vi "UI Subpanel.vi"() -> ()   [LabVIEW 2021, in "CIF CAN_Reader_CANsub UI.lvlib"]
uses:
  CIF CAN_Reader_CANsub UI.lvlib
  Common/Typedef/Configuration.ctl
  <vilib>/CIF Foundation/CIF Core/CIFCore/Common/Typedef/Common Plugin Configuration.ctl
  <vilib>/CIF Foundation/CIF Core/CIFCore/Common/Typedef/External Clock Config.ctl
  <vilib>/CIF Foundation/CIF CAN RW Core/typedef/CAN Port Configuration.ctl
  <vilib>/CIF Foundation/CIF CAN RW Core/typedef/CAN Mode.ctl
  <vilib>/CIF Foundation/CIF CAN RW Core/typedef/FD Config.ctl
  <vilib>/CIF Foundation/CIF CAN RW Core/typedef/CAN Filter.ctl
  <vilib>/CIF Foundation/CIF Core/CIFUI/Typedef/Class Data for SubPanel.ctl
  <vilib>/CIF Foundation/CIF Core/CIFUI/Typedef/Core UI References.ctl
  <vilib>/CIF Foundation/CIF Core/CIFUI/Typedef/Run Listen Button.ctl
  <vilib>/CIF Foundation/CIF Core/CIFUI/Typedef/SubPanel Events.ctl
  <vilib>/CIF Foundation/CIF Core/CIFUI/Typedef/New Connection Plugin Event Data.ctl
  Grpc/CanReaderCansub_client/RPC Messages/cif_can_reader_cansub_Statistics.ctl
  <vilib>/CIF Foundation/CIF CAN RW Core/typedef/CAN Status.ctl
  <vilib>/CIF Foundation/CIF CAN RW Core/typedef/Communication State.ctl
  <vilib>/CIF Foundation/CIF CAN RW Core/typedef/Last Error.ctl
  <vilib>/CIF Foundation/CIF Core/CIFUI/CIF_UI.lvclass
  <vilib>/CIF Foundation/CIF Core/CIFUI/CIF_UI.lvclass/CIF_UI.ctl
  <vilib>/CIF Foundation/CIF U8 Array Monitor gRPC/U8_Array_Monitor_gRPC/CIFU8ArrayMonitor_client/RPC Messages/cif_u8arraymonitor_SetEnableU8ArrayRequest.ctl
  <vilib>/CIF Foundation/CIF Core/CIFUI/Utilities/Get Human Readable Error.vi
  <vilib>/CIF Foundation/CIF Utilities/Errors/Append Error Location.vi
  <vilib>/CIF Foundation/CIF Utilities/Errors/Human Readable Error Message.vi
  Grpc/CAN_Reader_CANsub_wrapper/CAN_Reader_CANsub_Wrapper.lvlib
  <vilib>/addons/_JKI.lib/Serialization/JSON/JKI JSON Serialization.lvlib
  <vilib>/CIF Foundation/CIF Core/CIFCore/Grpc/CIFCoreWrapper/CIFCoreWrapper.lvlib
  <vilib>/CIF Foundation/CIF U8 Array Monitor gRPC/U8_Array_Monitor_gRPC/CIFU8ArrayMonitorWrapper/CIFU8ArrayMonitorWrapper.lvlib
  <vilib>/CIF Foundation/CIF U8 Array Monitor gRPC/U8_Array_Monitor_gRPC/CIFU8ArrayMonitor_client/CIFU8ArrayMonitor_client.lvlib
  <vilib>/CIF Foundation/CIF Core/CIFCore/Common/CIFCoreCommon.lvlib
  Common/CAN_Reader_CANsub_Common.lvlib
  <vilib>/CIF Foundation/CIF CAN RW Core/CAN_RW_CORE.lvclass
  Grpc/CanReaderCansub_client/CanReaderCansub_client.lvlib
panel:
  in  "Blink":bool
  in  "Refresh Device List":bool
  in  "Get CAN Data":bool
  in  "History":u32=10
  in  "Enable CAN Monitor":bool
  in  "Update Config":bool
  out "CAN Status":T1
  out "Devices":string[](array[string])
  out "Statistics":T4
  in  "Class Data for SubPanel":T5
  in  "Configuration":T8={"Common"={"Period (s)"=0.001, "Offset (us)"=0, "Priority"=100, "Processor"=-2, "External Clock"={"ClockID"=0, "Clock Name"="", "Publish Clock"=FALSE, "Convert Data Timestamps"=FALSE, "Plugin Timing Source"=FALSE}}, "RX Interface"="CAN2", "Port Configuration"={"Mode"=enum."CAN FD", "Baud Rate"=500000, "Temination On"=TRUE, "Subordinate"=FALSE, "Echo TX"=FALSE, "FD Config"={"FD Baud Rate"=2000000, "ISO Mode"=TRUE, "BRS Enabled"=TRUE}}, "Timeout (ms)"=100, "Frames to read"=100, "Filter"={"Allow List (ID)"=[], "Deny List (ID)"=[]}} {"Filter"."Deny List (ID)" format="%.0x"; "Filter"."Allow List (ID)" format="%.0x"; "Port Configuration"."FD Config"."FD Baud Rate" format="%.0p"; "Port Configuration"."Baud Rate" format="%.0p"; "Common"."Period (s)" format="%#_13g"}
  out "Plugin Status":string[][](table)
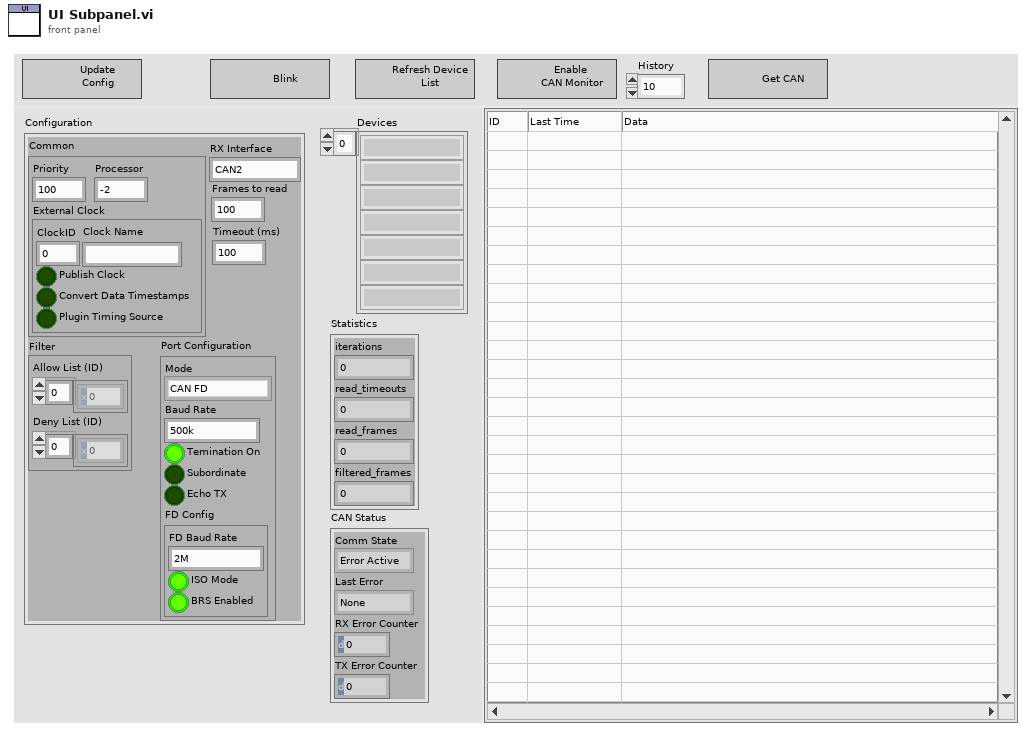
[diagram p1: front panel]
types:
  T1 = typedef "CAN_RW_CORE.lvclass/CAN Status.ctl" = cluster{"Comm State":T2, "Last Error":T3, "RX Error Counter":u8, "TX Error Counter":u8}
  T2 = typedef "CAN_RW_CORE.lvclass/Communication State.ctl" = enum16{"Error Active", "Error Passive", "Bus Off"}
  T3 = typedef "CAN_RW_CORE.lvclass/Last Error.ctl" = enum16{"None", "Stuff", "Form", "Ack", "Bit1", "Bit0", "CRC", "Unknown"}
  T4 = typedef "CanReaderCansub_client.lvlib/cif_can_reader_cansub_Statistics.ctl" = cluster{"iterations":u64, "read_timeouts":u64, "read_frames":u64, "filtered_frames":u64}
  T5 = typedef "CIF_UI.lvclass/Class Data for SubPanel.ctl" = cluster{"IP Address":string, "Server Certificate File (.crt)":path, "Connected":bool, "Core UI References":T6, "Subpanel Events":T7, "Manager gRPC Port":u16}
  T6 = typedef "CIF_UI.lvclass/Core UI References.ctl" = cluster{"Plugin Status":refnum<vi>, "Plugin Status Valid":bool, "Connection":refnum<vi>, "Connection Valid":bool, "Exit":refnum<vi>, "Exit Valid":bool, "Run Listen":refnum<vi>, "Run Listen Valid":bool, "Clear Local Error":refnum<vi>, "Clear Local Error Valid":bool, "Local Error":refnum<vi>, "Local Error Valid":bool}
  T7 = typedef "CIF_UI.lvclass/SubPanel Events.ctl" = cluster{"Clear Local Error":refnum<user-event>, "Shutdown":refnum<user-event>, "Plugin Connection":refnum<user-event>}
  T8 = typedef "CAN_Reader_CANsub_Common.lvlib/Configuration.ctl" = cluster{"Common":T9, "RX Interface":string, "Port Configuration":T11, "Timeout (ms)":i32, "Frames to read":i32, "Filter":T14}
  T9 = typedef "CIFCoreCommon.lvlib/Common Plugin Configuration.ctl" = cluster{"Period (s)":dbl, "Offset (us)":i32, "Priority":i32, "Processor":i32, "External Clock":T10}
  T10 = typedef "CIFCoreCommon.lvlib/External Clock Config.ctl" = cluster{"ClockID":u8, "Clock Name":string, "Publish Clock":bool, "Convert Data Timestamps":bool, "Plugin Timing Source":bool}
  T11 = typedef "CAN_RW_CORE.lvclass/CAN Port Configuration.ctl" = cluster{"Mode":T12, "Baud Rate":u64, "Temination On":bool, "Subordinate":bool, "Echo TX":bool, "FD Config":T13}
  T12 = typedef "CAN_RW_CORE.lvclass/CAN Mode.ctl" = enum16{"CAN 2.0", "CAN FD"}
  T13 = typedef "CAN_RW_CORE.lvclass/FD Config.ctl" = cluster{"FD Baud Rate":u64, "ISO Mode":bool, "BRS Enabled":bool}
  T14 = typedef "CAN_RW_CORE.lvclass/CAN Filter.ctl" = cluster{"Allow List (ID)":u32[], "Deny List (ID)":u32[]}
  T15 = typedef "grpc-lvsupport-release.lvlib/grpcId.ctl" = u64
  T16 = typedef "CIFU8ArrayMonitor_client.lvlib/cif_u8arraymonitor_SetEnableU8ArrayRequest.ctl" = cluster{"enable_u8_array":bool, "history_depth":u32}
  T17 = typedef "CanReaderCansub_client.lvlib/cif_can_reader_cansub_CansubDevice.ctl" = cluster{"interface":string, "slot":u32, "device_id":string}
  T18 = typedef "CAN_Reader_NIXNET_Common.lvlib/Configuration.ctl" = cluster{"Common":T9, "RX Interface":string, "Port Configuration":T11, "Timeout (ms)":i32, "Frames to read":i32, "Filter":T14}
  T19 = typedef "CIFU8ArrayMonitor_client.lvlib/cif_u8arraymonitor_U8Arrays.ctl" = cluster{"u8_array":T20[], "valid":bool}
  T20 = typedef "CIFU8ArrayMonitor_client.lvlib/cif_u8arraymonitor_U8Array.ctl" = cluster{"u8_array":u8[], "timestamp":i64}
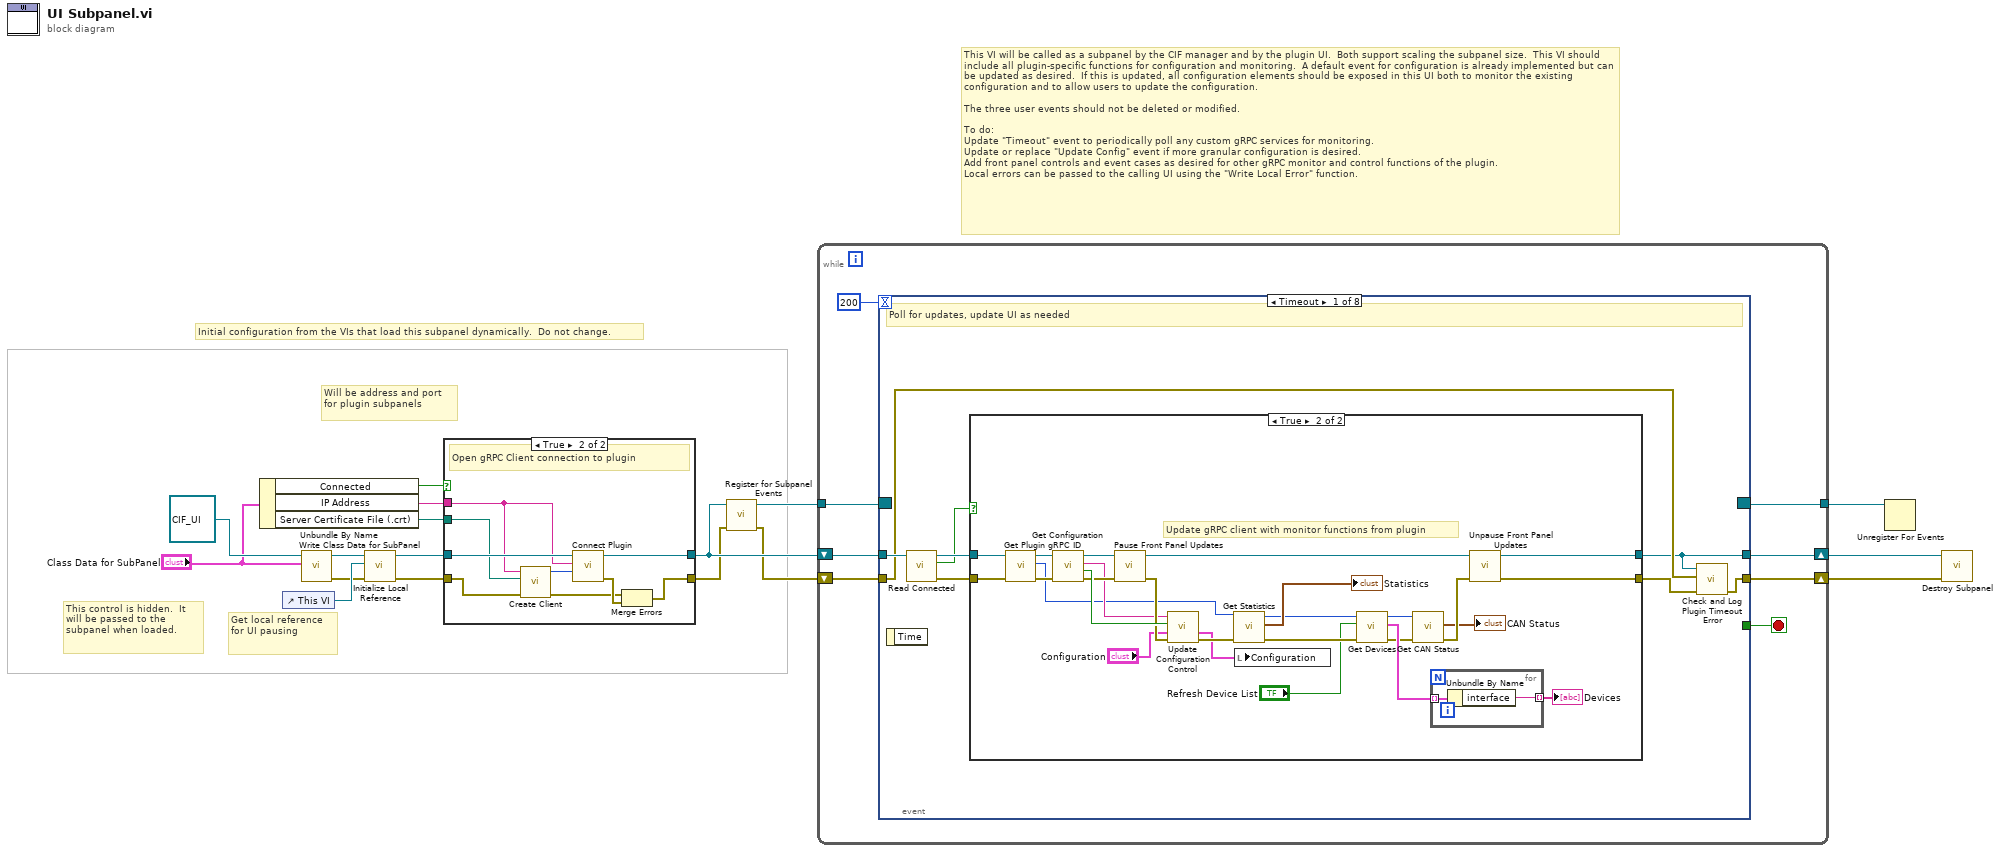
[diagram p0: block diagram]
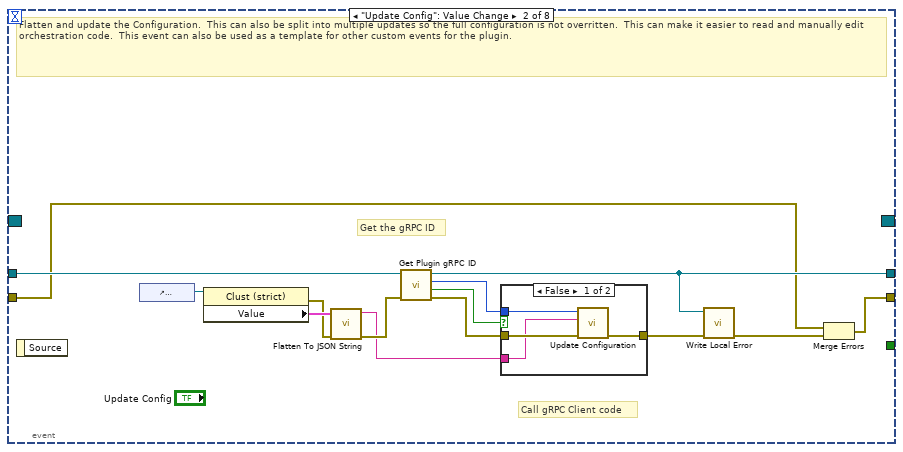
[diagram p4: hidden frame]
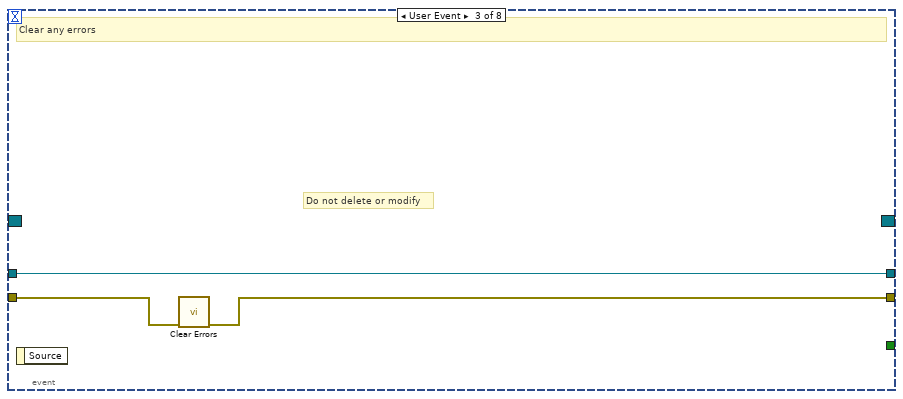
[diagram p6: hidden frame]
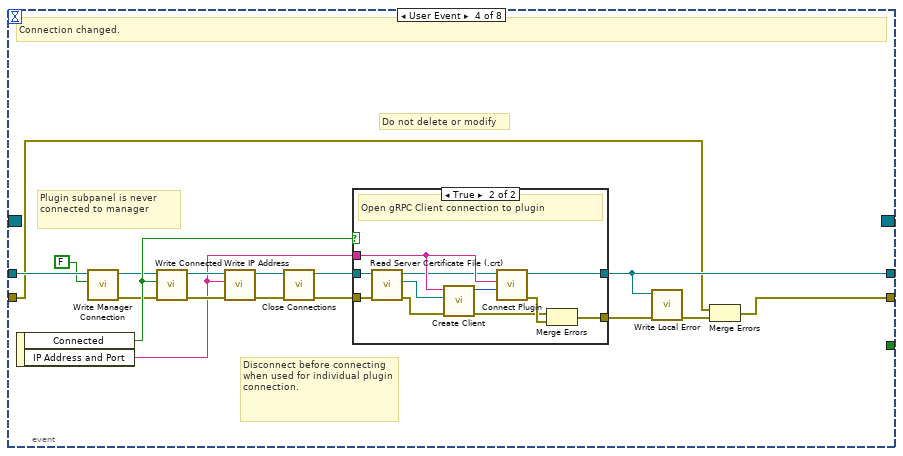
[diagram p7: hidden frame]
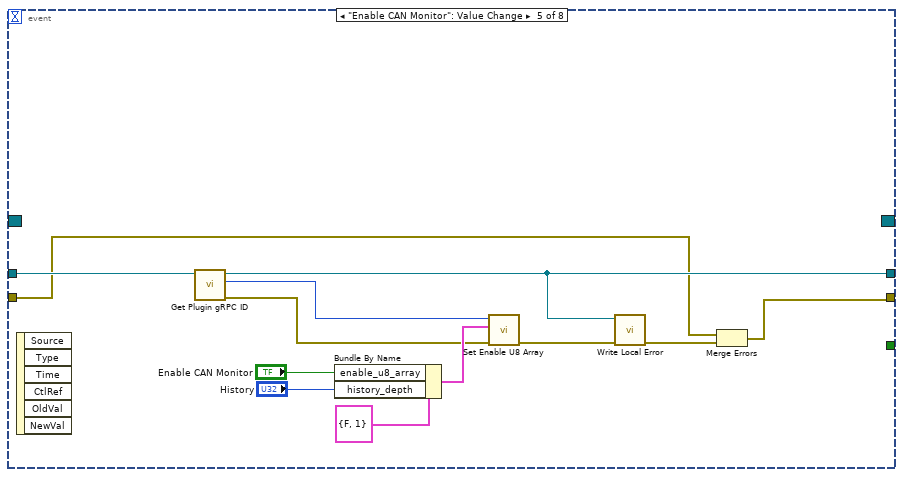
[diagram p9: hidden frame]
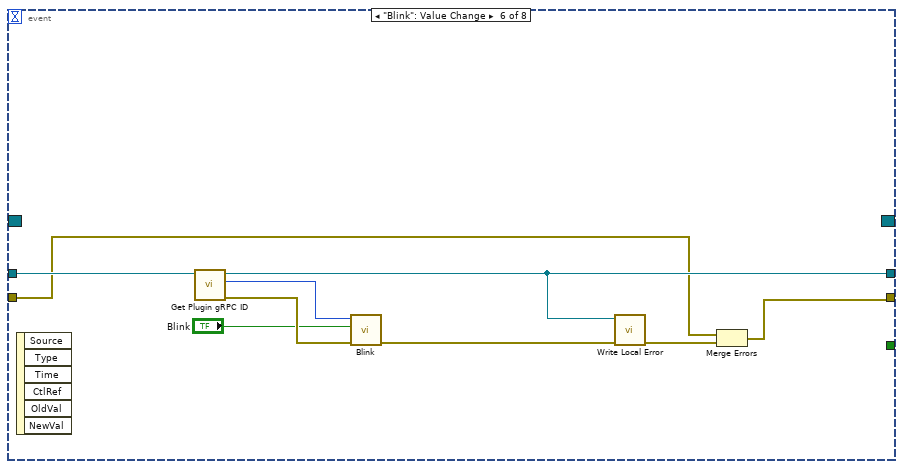
[diagram p10: hidden frame]
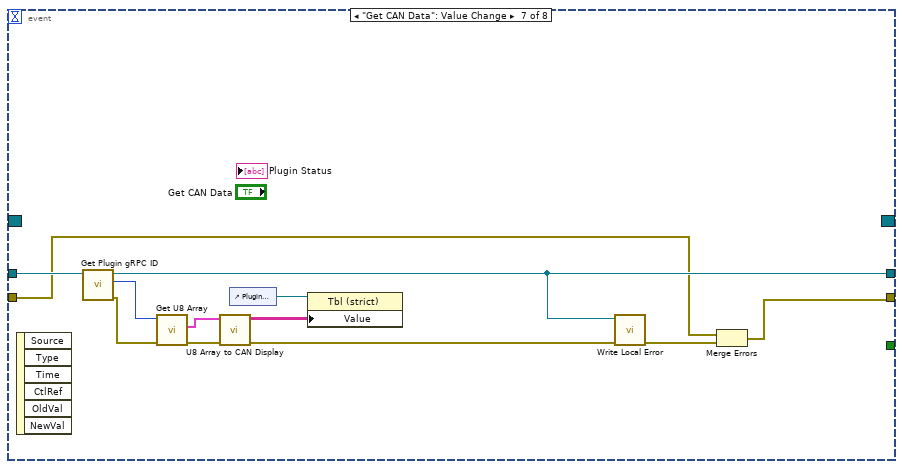
[diagram p11: hidden frame]
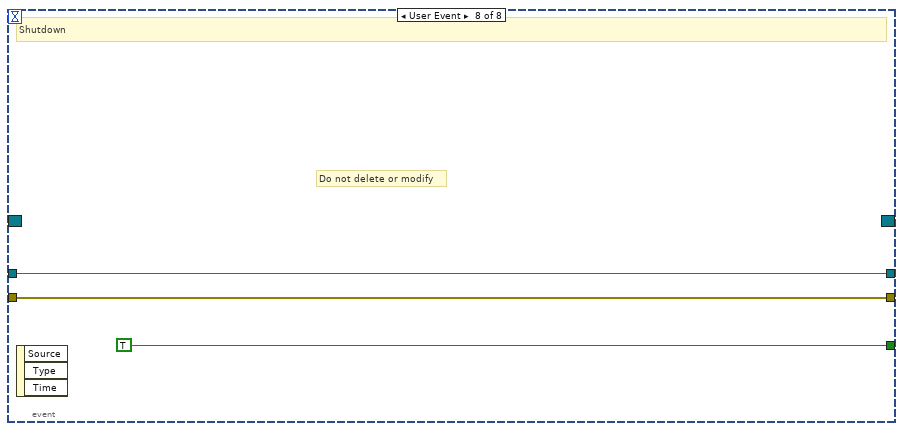
[diagram p12: hidden frame]
diagram:
  # "Initial configuration from the VIs that load this subpanel dynamically.  Do not change."
  # "This control is hidden.  It will be passed to the subpanel when loaded."
  # "This VI will be called as a subpanel by the CIF manager and by the plugin UI.  Both support scaling the subpanel size.  This VI should include all plugin-specific functions for configuration and monitoring.  A default event for configuration is already implemented but can be updated as desired.  If this is updated, all configuration elements should be exposed in this UI both to monitor the existing configuration and to allow users to update the configuration.\n\nThe three user events should not be deleted or modified.\n\nTo do:\nUpdate \"Timeout\" event to periodically poll any custom gRPC services for monitoring.\nUpdate or replace \"Update Config\" event if more granular configuration is desired.\nAdd front panel controls and event cases as desired for other gRPC monitor and control functions of the plugin.\nLocal errors can be passed to the calling UI using the \"Write Local Error\" function."
  # "Will be address and port for plugin subpanels"
  # "Get local reference for UI pausing"
  n1 = Unbundle By Name("Class Data for SubPanel") -> ("Connected"=w8:bool, "IP Address"=w7:string, "Server Certificate File (.crt)"=w6:path)
  n2 = control-ref of="This VI"() -> (w17:refnum<vi>)
  n3 = call <vilib>:"Write Class Data for SubPanel.vi"("Class Data for SubPanel"="Class Data for SubPanel", "CIF_UI in"=refnum<class "CIF_UI.lvclass"> refnum) -> ("error out"=w12:errorcluster, "CIF_UI out"=w14:refnum<class "CIF_UI.lvclass">)  [unwired: 8 in]
  n4 = call <vilib>:"Initialize Local Reference.vi"("error in (no error)"=w12, "This VI"=w17, "CIF_UI in"=w14) -> ("error out"=w10:errorcluster, "CIF_UI out"=w11:refnum<class "CIF_UI.lvclass">)  [unwired: 7 in]
  n5 = case shown="True" w8 {
    tunnel: [w18 w28] -> w4
    tunnel: [w19 w26] -> w5
    tunnel: w11 -> [w19 w25]
    tunnel: w10 -> [w18 w24]
    tunnel: w7 -> [_ w21]
    tunnel: w6 -> [_ w20]
    frame False {
    }
    frame True {
      # "Open gRPC Client connection to plugin"
      n6 = call "Create Client.vi"("error in"=w24, "Server Certificate File (.crt)"=w20, "address"=w21) -> ("error out"=w23:errorcluster, "gRPC ID Out"=w22:T15)  [unwired: 7 in]
      n7 = call <vilib>:"Connect Plugin.vi"("gRPC ID"=w22, "Address"=w21, "CIF_UI in"=w25) -> ("error out"=w27:errorcluster, "CIF_UI out"=w26:refnum<class "CIF_UI.lvclass">)  [unwired: 7 in]
      n8 = Merge Errors(w23, w27) -> (w28:errorcluster)
    }
  }
  n9 = call <vilib>:"Register for Subpanel Events.vi"("error in (no error)"=w4, "CIF_UI in"=w5) -> ("error out"=w2:errorcluster, "Event Registration Refnum"=w3:refnum<event-registration>)  [unwired: 8 in]
  n10 = while {
    tunnel: w3 -> [w35]
    shift-right: [w30] -> w16
    shift-left: w5 -> [w33]
    shift-right: [w31] -> w1
    shift-left: w2 -> [w32]
    tunnel: [w29] -> w15
    stop <- w34 stop-if-true
    n11 = event shown="[0] Timeout" {
      selector: w35 -> [_ _ _ _ _ _ _ _]
      dyn-events: [_ _ _ _ _ _ _ _] -> w29
      timeout: 200 -> [_ _ _ _ _ _ _ _]
      tunnel: [_ _ _ _ _ _ _ TRUE] -> w34
      tunnel: w33 -> [w41 w85 w94 w105 w137 w146 w158 w161]
      tunnel: w32 -> [w38 w79 w96 w98 w135 w144 w156 w160]
      tunnel: [w39 w78 w95 w97 w134 w143 w155 w160] -> w31
      tunnel: [w37 w81 w94 w99 w136 w145 w157 w161] -> w30
      event Timeout {
        # "Poll for updates, update UI as needed"
        n12 = event-data() -> ()  [unwired: 1 in, 1 out]
        n13 = call <vilib>:"Read Connected.vi"("CIF_UI in"=w41) -> ("error out"=w43:errorcluster, "Connected"=w42:bool, "CIF_UI out"=w44:refnum<class "CIF_UI.lvclass">)  [unwired: 8 in]
        n14 = case shown="True" w42 {
          tunnel: w43 -> [w45 w64]
          tunnel: [w45 w72] -> w40
          tunnel: w44 -> [w46 w65]
          tunnel: [w46 w71] -> w37
          frame False {
          }
          frame True {
            # "Update gRPC client with monitor functions from plugin"
            n15 = call <vilib>:"Get Plugin gRPC ID.vi"("error in (no error)"=w64, "CIF_UI in"=w65) -> ("error out"=w62:errorcluster, "gRPC ID"=w59:T15, "CIF_UI out"=w63:refnum<class "CIF_UI.lvclass">)  [unwired: 5 in, 2 out]
            n16 = call <vilib>:"Get Configuration.vi"("error in (no error)"=w62, "CIF_Plugin_UI in"=w63) -> ("error out"=w68:errorcluster, "Not Found"=w70:bool, "JSON Configuration"=w61:string, "CIF_Plugin_UI out"=w69:refnum<class "CIF_UI.lvclass">)  [unwired: 6 in]
            n17 = call <vilib>:"Pause Front Panel Updates.vi"("error in (no error)"=w68, "CIF_UI in"=w69) -> ("error out"=w67:errorcluster, "CIF_UI out"=w66:refnum<class "CIF_UI.lvclass">)  [unwired: 8 in]
            n18 = call "Update Configuration Control.vi"("error in (no error)"=w67, "Configuration in"="Configuration", "Not Valid"=w70, "JSON Configuration"=w61) -> ("error out"=w60:errorcluster, "Configuration out"=w56:T8)  [unwired: 6 in]
            n19 = call "Get Statistics.vi"("error in"=w60, "gRPC ID"=w59) -> ("error out"=w55:errorcluster, "Statistics"=→"Statistics":T4, "gRPC ID out"=w53:T15)  [unwired: 7 in]
            n20 = local write "Configuration"(w56) -> ()
            n21 = call "Get Devices.vi"("error in"=w55, "Refresh Device List"="Refresh Device List", "gRPC ID"=w53) -> ("error out"=w50:errorcluster, "devices"=w52:T17[], "gRPC ID out"=w49:T15)  [unwired: 6 in]
            n22 = call "Get CAN Status.vi"("error in"=w50, "gRPC ID"=w49) -> ("error out"=w48:errorcluster, "CAN Status"=→"CAN Status":T1)  [unwired: 7 in, 1 out]
            n23 = for {
              tunnel: w52 -> [w74] mode=indexing
              tunnel: [w73] -> w51 mode=indexing
              n24 = Unbundle By Name(w74) -> ("interface"=w73:string)
            }
            "Devices" <- w51
            n25 = call <vilib>:"Unpause Front Panel Updates.vi"("error in (no error)"=w48, "CIF_UI in"=w66) -> ("error out"=w72:errorcluster, "CIF_UI out"=w71:refnum<class "CIF_UI.lvclass">)  [unwired: 8 in]
          }
        }
        n26 = call <vilib>:"Check and Log Plugin Timeout Error.vi"("New Error"=w40, "Previous Error"=w38, "CIF_UI in"=w37) -> ("error out"=w39:errorcluster)  [unwired: 8 in]
      }
      event "Update Config": Value Change {
        # "Call gRPC Client code"
        # "Get the gRPC ID"
        # "Flatten and update the Configuration.  This can also be split into multiple updates so the full configuration is not overritten.  This can make it easier to read and manually edit orchestration code.  This event can also be used as a template for other custom events for the plugin."
        n27 = event-data() -> ()  [unwired: 1 in, 1 out]
        n28 = control-ref of="Configuration"() -> (w77:refnum<vi>)
        n29 = property class="Clust (strict)"(reference=w77) -> (error out=w75:errorcluster, "Value"=w76:T18)  [unwired: 1 in, 1 out]
        n30 = call <vilib>:"Flatten To JSON String.vi"("error in"=w75, "Variant"=w76) -> ("error out"=w84:errorcluster, "JSON String"=w83:string)  [unwired: 8 in]
        n31 = call <vilib>:"Get Plugin gRPC ID.vi"("error in (no error)"=w84, "CIF_UI in"=w85) -> ("error out"=w86:errorcluster, "Not Found"=w87:bool, "gRPC ID"=w88:T15, "CIF_UI out"=w81:refnum<class "CIF_UI.lvclass">)  [unwired: 5 in, 1 out]
        n32 = case shown="False" w87 {
          tunnel: w88 -> [w92 _]
          tunnel: w86 -> [w91 w93]
          tunnel: [w90 w93] -> w82
          tunnel: w83 -> [w89 _]
          frame False {
            n33 = call <vilib>:"Update Configuration.vi"("error in"=w91, "JSON Configuration"=w89, "gRPC ID"=w92) -> ("error out"=w90:errorcluster)  [unwired: 7 in, 1 out]
          }
          frame True {
          }
        }
        n34 = call <vilib>:"Write Local Error.vi"("error in (no error)"=w82, "CIF_UI in"=w81) -> ("error out"=w80:errorcluster)  [unwired: 9 in]
        n35 = Merge Errors(w79, w80) -> (w78:errorcluster)
      }
      event User Event {
        # "Do not delete or modify"
        # "Clear any errors"
        n36 = event-data() -> ()  [unwired: 1 in, 1 out]
        n37 = call <vilib>:"Clear Errors.vi"("error in (no error)"=w96) -> ("error out"=w95:errorcluster)  [unwired: 5 in, 1 out]
      }
      event User Event {
        # "Do not delete or modify"
        # "Plugin subpanel is never connected to manager"
        # "Disconnect before connecting when used for individual plugin connection."
        # "Connection changed."
        n38 = event-data() -> ("Connected"=w106:bool, "IP Address and Port"=w107:string)  [unwired: 1 in]
        n39 = call <vilib>:"Write Manager Connection.vi"("Manager Connection"=FALSE, "CIF_UI in"=w105) -> ("error out"=w103:errorcluster, "CIF_UI out"=w104:refnum<class "CIF_UI.lvclass">)  [unwired: 8 in]
        n40 = call <vilib>:"Write Connected.vi"("error in (no error)"=w103, "Connected"=w106, "CIF_UI in"=w104) -> ("error out"=w112:errorcluster, "CIF_UI out"=w113:refnum<class "CIF_UI.lvclass">)  [unwired: 7 in]
        n41 = call <vilib>:"Write IP Address.vi"("error in (no error)"=w112, "IP Address"=w107, "CIF_UI in"=w113) -> ("error out"=w110:errorcluster, "CIF_UI out"=w111:refnum<class "CIF_UI.lvclass">)  [unwired: 7 in]
        n42 = call <vilib>:"Close Connections.vi"("error in (no error)"=w110, "CIF_UI in"=w111) -> ("error out"=w108:errorcluster, "CIF_UI out"=w109:refnum<class "CIF_UI.lvclass">)  [unwired: 8 in]
        n43 = case shown="True" w106 {
          tunnel: [w114 w126] -> w100
          tunnel: [w115 w124] -> w99
          tunnel: w109 -> [w115 w120]
          tunnel: w108 -> [w114 w119]
          tunnel: w107 -> [_ w121]
          frame False {
          }
          frame True {
            # "Open gRPC Client connection to plugin"
            n44 = call <vilib>:"Read Server Certificate File (.crt).vi"("error in (no error)"=w119, "CIF_UI in"=w120) -> ("error out"=w117:errorcluster, "Server Certificate File (.crt)"=w116:path, "CIF_UI out"=w118:refnum<class "CIF_UI.lvclass">)  [unwired: 7 in]
            n45 = call "Create Client.vi"("error in"=w117, "Server Certificate File (.crt)"=w116, "address"=w121) -> ("error out"=w123:errorcluster, "gRPC ID Out"=w122:T15)  [unwired: 7 in]
            n46 = call <vilib>:"Connect Plugin.vi"("gRPC ID"=w122, "Address"=w121, "CIF_UI in"=w118) -> ("error out"=w125:errorcluster, "CIF_UI out"=w124:refnum<class "CIF_UI.lvclass">)  [unwired: 7 in]
            n47 = Merge Errors(w123, w125) -> (w126:errorcluster)
          }
        }
        n48 = call <vilib>:"Write Local Error.vi"("error in (no error)"=w100, "CIF_UI in"=w99) -> ("error out"=w101:errorcluster)  [unwired: 9 in]
        n49 = Merge Errors(w98, w101) -> (w97:errorcluster)
      }
      event "Enable CAN Monitor": Value Change {
        n50 = event-data() -> ()  [unwired: 1 in, 6 out]
        n51 = call <vilib>:"Get Plugin gRPC ID.vi"("CIF_UI in"=w137) -> ("error out"=w129:errorcluster, "gRPC ID"=w133:T15, "CIF_UI out"=w136:refnum<class "CIF_UI.lvclass">)  [unwired: 6 in, 2 out]
        n52 = Bundle By Name(cluster=T16 {"enable_u8_array"=FALSE, "history_depth"=1} ("Enable Request"), "enable_u8_array"="Enable CAN Monitor", "history_depth"="History") -> (w130:T16)
        n53 = call <vilib>:"Set Enable U8 Array.vi"("error in"=w129, "Enable Request"=w130, "gRPC ID"=w133) -> ("error out"=w128:errorcluster)  [unwired: 7 in, 1 out]
        n54 = call <vilib>:"Write Local Error.vi"("error in (no error)"=w128, "CIF_UI in"=w136) -> ("error out"=w138:errorcluster)  [unwired: 9 in]
        n55 = Merge Errors(w135, w138) -> (w134:errorcluster)
      }
      event "Blink": Value Change {
        n56 = event-data() -> ()  [unwired: 1 in, 6 out]
        n57 = call <vilib>:"Get Plugin gRPC ID.vi"("CIF_UI in"=w146) -> ("error out"=w141:errorcluster, "gRPC ID"=w142:T15, "CIF_UI out"=w145:refnum<class "CIF_UI.lvclass">)  [unwired: 6 in, 2 out]
        n58 = call "Blink.vi"("error in"=w141, "blink"="Blink", "gRPC ID"=w142) -> ("error out"=w140:errorcluster)  [unwired: 7 in, 1 out]
        n59 = call <vilib>:"Write Local Error.vi"("error in (no error)"=w140, "CIF_UI in"=w145) -> ("error out"=w147:errorcluster)  [unwired: 9 in]
        n60 = Merge Errors(w144, w147) -> (w143:errorcluster)
      }
      event "Get CAN Data": Value Change {
        n61 = event-data() -> ()  [unwired: 1 in, 6 out]
        n62 = call <vilib>:"Get Plugin gRPC ID.vi"("CIF_UI in"=w158) -> ("error out"=w153:errorcluster, "gRPC ID"=w154:T15, "CIF_UI out"=w157:refnum<class "CIF_UI.lvclass">)  [unwired: 6 in, 2 out]
        n63 = call <vilib>:"Get U8 Array.vi"("error in"=w153, "gRPC ID"=w154) -> ("error out"=w151:errorcluster, "U8 Array"=w152:T19)  [unwired: 7 in, 1 out]
        n64 = call "U8 Array to CAN Display.vi"("error in (no error)"=w151, "U8 Array"=w152) -> ("error out"=w150:errorcluster, "CAN Data for Mutli Listbox"=w148:string[][])  [unwired: 8 in]
        n65 = control-ref of="Plugin Status"() -> (w149:refnum<vi>)
        n66 = property class="Tbl (strict)"(reference=w149, "Value"=w148) -> ()  [unwired: 1 in, 2 out]
        n67 = call <vilib>:"Write Local Error.vi"("error in (no error)"=w150, "CIF_UI in"=w157) -> ("error out"=w159:errorcluster)  [unwired: 9 in]
        n68 = Merge Errors(w156, w159) -> (w155:errorcluster)
      }
      event User Event {
        # "Do not delete or modify"
        # "Shutdown"
        n69 = event-data() -> ()  [unwired: 1 in, 3 out]
      }
    }
  }
  n70 = Unregister For Events(event registration refnum=w15) -> ()  [unwired: 1 in, 1 out]
  n71 = call <vilib>:"Destroy Subpanel.vi"("error in (no error)"=w1, "CIF_UI in"=w16) -> ()  [unwired: 8 in, 2 out]
